vi "set Measurement Window Mode - FSV40.vi"(8 "error in (no error)":errorcluster, 10 "Measurement Window Mode":T1, 11 "Interface_Spectrum in":refnum<class "Interface_Spectrum.lvclass">) -> (0 "error out":errorcluster, 3 "Interface_Spectrum out":refnum<class "Interface_Spectrum.lvclass">)   [LabVIEW 2023, in "Spectrum Analyzer.lvlib" / "Interface_Spectrum.lvclass"]
doc: "1) ACPower\nAdjacent-channel power measurement with a single carrier signal\n2) CPOWer\nChannel power measurement with a single carrier signal (equivalent to adjacent-channel power measurement with \"NO. OF ADJ CHAN\" = 0)\n3) MCACpower\nChannel/adjacent-channel power measurement with several carrier signals\n4) OBANdwidth | OBWidth\nMeasurement of occupied bandwidth\n5) CN\nMeasurement of carrier-to-noise ratio\n6) CN0\nMeasurement of carrier-to-noise ratio referenced to 1 Hz bandwidth"
uses:
  Interface_Spectrum.lvclass
  TYPE DEFINITION/TYPE Measurement Window Mode.ctl
  Spectrum Analyzer.lvlib
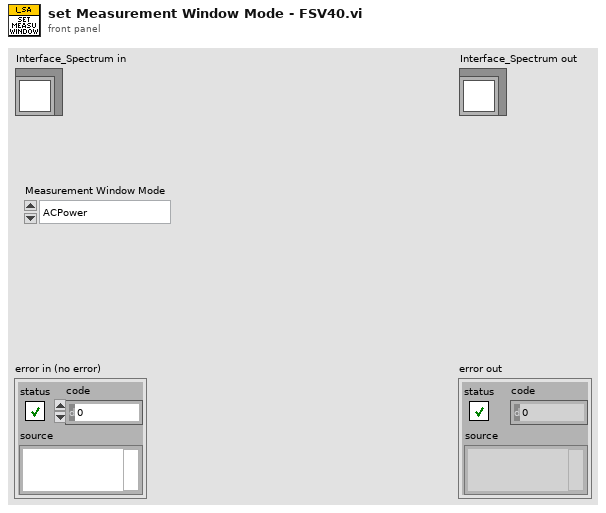
[diagram p1: front panel]
types:
  T1 = typedef "Spectrum Analyzer.lvlib/TYPE Measurement Window Mode.ctl" = enum16{"ACPower", "CPOWer", "MCACpower", "OBANdwidth", "OBWidth", "CN", "CN0"}
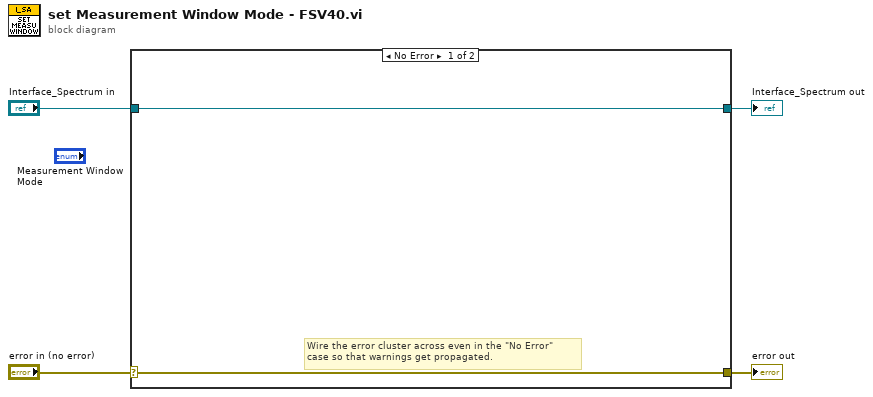
[diagram p0: block diagram]
diagram:
  n1 = case shown="No Error" "error in (no error)" {
    selector: "error in (no error)" -> [w5 w8]
    tunnel: [w5 w8] -> w3
    tunnel: [w6 w7] -> w1
    tunnel: "Interface_Spectrum in" -> [w6 w7]
    frame No Error {
      # "Wire the error cluster across even in the \"No Error\"\ncase so that warnings get propagated."
    }
    frame Error {
    }
  }
  "error out" <- w3
  "Interface_Spectrum out" <- w1
